vi "search Max Index.vi"(0 "Trace Values":T1 {"Frequency" format="%#_6p"}, 1 "Search Range":cluster{"Start":dbl, "End":dbl}) -> (8 "Index":i32)   [LabVIEW 2023, in "Instrument Manager.lvclass"]
uses:
  Instrument Manager.lvclass
  Module/Spectrum Analyzer/TYPE DEFINITION/TYPE Trace Value Array.ctl
  Instrument Manager.lvclass/Instrument Manager.ctl
  Module/Spectrum Analyzer/Spectrum Analyzer.lvlib
panel:
  out "크기":i32
  out "x-y":i32
  out "원소의 인덱스 3":i32
  out "Amplitude":dbl[](array[numeric])
  out "최소(x,y)":i32
  out "원소의 인덱스":i32
  out "최대 인덱스":i32
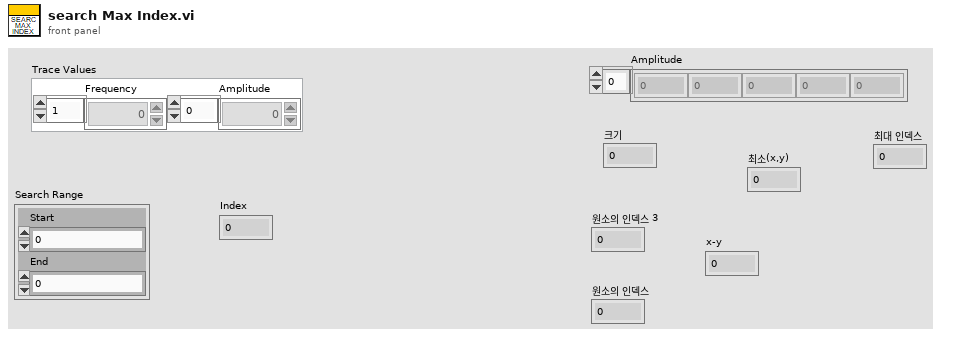
[diagram p1: front panel]
types:
  T1 = typedef "Spectrum Analyzer.lvlib/TYPE Trace Value Array.ctl" = cluster{"Frequency":dbl[], "Amplitude":dbl[]}
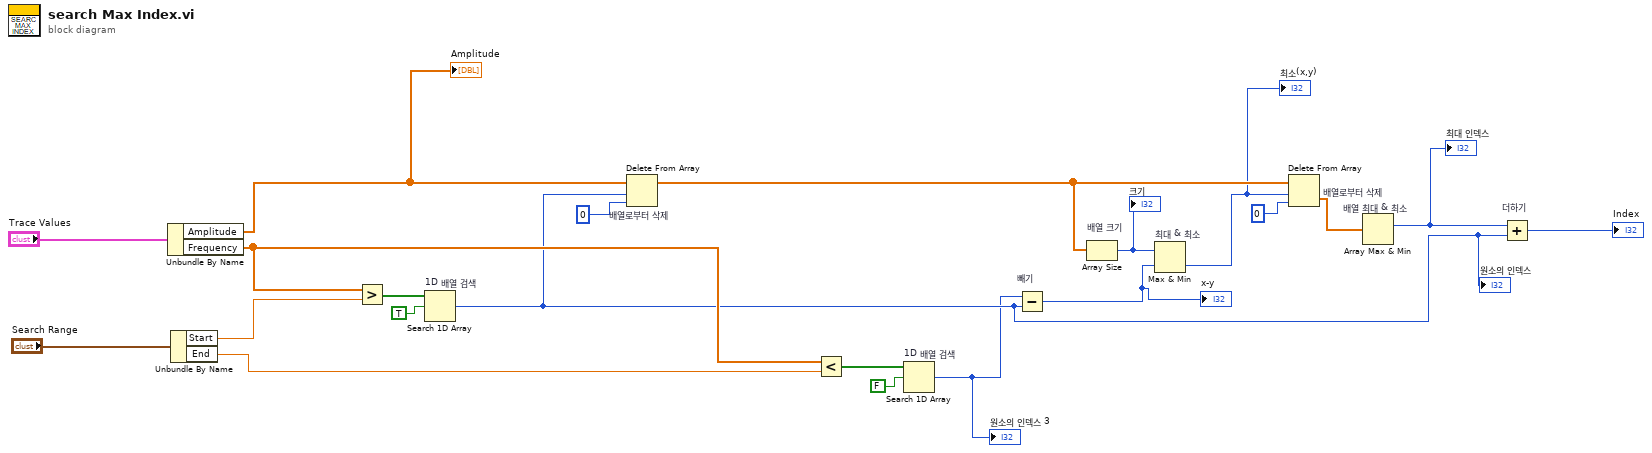
[diagram p0: block diagram]
diagram:
  n1 = Unbundle By Name("Trace Values") -> ("Amplitude"=w7:dbl[], "Frequency"=w10:dbl[])
  "Amplitude" <- w7
  n2 = Unbundle By Name("Search Range") -> ("Start"=w12:dbl, "End"=w11:dbl)
  n3 = Greater?(x=w10, y=w12) -> (0:w2:bool[])
  n4 = Search 1D Array "1D 배열 검색"(1D array=w2, element=TRUE ("원소")) -> (index of element=w6:i32)  [unwired: 1 in]
  "원소의 인덱스" <- w6
  n5 = Delete From Array "배열로부터 삭제"(array=w7, length=w6, index=0 ("인덱스")) -> (array with subset deleted=w17:dbl[])  [unwired: 1 out]
  n6 = Less?(x=w10, y=w11) -> (x < y?=w1:bool[])
  n7 = Search 1D Array "1D 배열 검색"(1D array=w1, element=FALSE ("원소")) -> (index of element=w5:i32)  [unwired: 1 in]
  "원소의 인덱스 3" <- w5
  n8 = Subtract "빼기"(x=w5, y=w6) -> (x-y=w4:i32)
  "x-y" <- w4
  n9 = Array Size "배열 크기"(array=w17) -> (size(s)=w3:i32)
  "크기" <- w3
  n10 = Max & Min "최대 & 최소"(x=w3, y=w4) -> (min(x,y)=w8:i32)  [unwired: 1 out]
  "최소(x,y)" <- w8
  n11 = Delete From Array "배열로부터 삭제"(array=w17, length=w8, index=0 ("인덱스")) -> (deleted portion=w15:dbl[])  [unwired: 1 out]
  n12 = Array Max & Min "배열 최대 & 최소"(array=w15) -> (max index (indices)=w9:i32)  [unwired: 3 out]
  "최대 인덱스" <- w9
  n13 = Add "더하기"(x=w9, y=w6) -> (x+y=→"Index":i32)
